vi "Edit_Sub_ConvertConfigFileDataToListItems.vi"(10 "Property":T1[](array[typedef]), 11 "Label":string) -> (3 "Array":string[](array[string]))   [LabVIEW 2019, in "Language Editor.lvlib"]
doc: "Konvertiere die Daten aus der Ini, sodass diese im UI angezeigt werden können.\n- - -\nCopyright (c) 2026, Merecs Engineering GmbH"
uses:
  Language Editor.lvlib
  Language Selection/TypeDefs/Cluster PropertyTranslation.ctl
  Language Selection/TypeDefs/Enum Property Type.ctl
  Language Selection/Language Selection.lvlib
panel:
  # "Connector Pane"
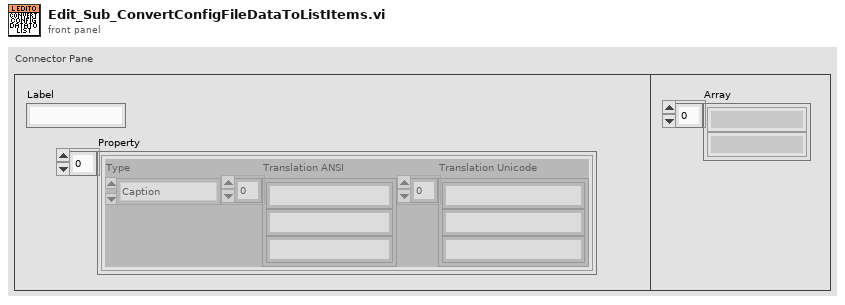
[diagram p1: front panel]
types:
  T1 = typedef "Language Selection.lvlib/Cluster PropertyTranslation.ctl" = cluster{"Type":T2, "Translation ANSI":string[], "Translation Unicode":string[]}
  T2 = typedef "Language Selection.lvlib/Enum Property Type.ctl" = enum16{"NA", "Caption", "String Value", "Boolean Text", "Ring Strings", "1D Array Elements", "2D Array Elements", "(MC)Listbox Header", "(MC)Listbox Items", "Tab Pages Names", "X & Y GraphChart", "Plot Names", "Table Headers", "Table Items", "TipStrip", "Combobox Strings", "Cursor Name", "Tree Col Headers"}
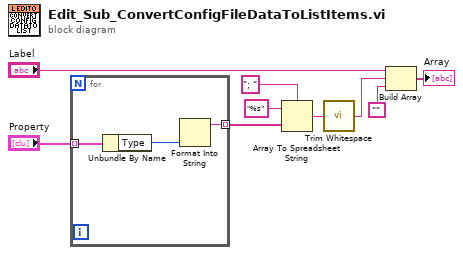
[diagram p0: block diagram]
diagram:
  n1 = for {
    tunnel: "Property" -> [w12] mode=indexing
    tunnel: [w10] -> w5 mode=indexing
    n2 = Unbundle By Name(w12) -> ("Type"=w11:T2)
    n3 = Format Into String(w11) -> (resulting string=w10:string)  [unwired: 3 in, 1 out]
  }
  n4 = Array To Spreadsheet String(delimiter (Tab)="; ", array=w5, 3:"%s" ("format string")) -> (spreadsheet string=w6:string)
  n5 = call <vilib>:"Trim Whitespace.vi"("string"=w6) -> ("trimmed string"=w8:string)  [unwired: 1 in]
  n6 = Build Array("Label", w8, "") -> (→"Array":string[])
